vi "LSignal Numbering.vi"(8 "Signal Tag A":string[](array[string]), 9 "Selected L#":i32[](array[numeric]), 10 "Selected S IDX":i32[](array[numeric]), 11 "Signal Profile Table A":string[][](table) caption="Singla Profile Table") -> (0 "BS Table":string[][](table) caption="Singla Profile Table", 3 "L# for T":i32[](array[numeric]))   [LabVIEW 2018]
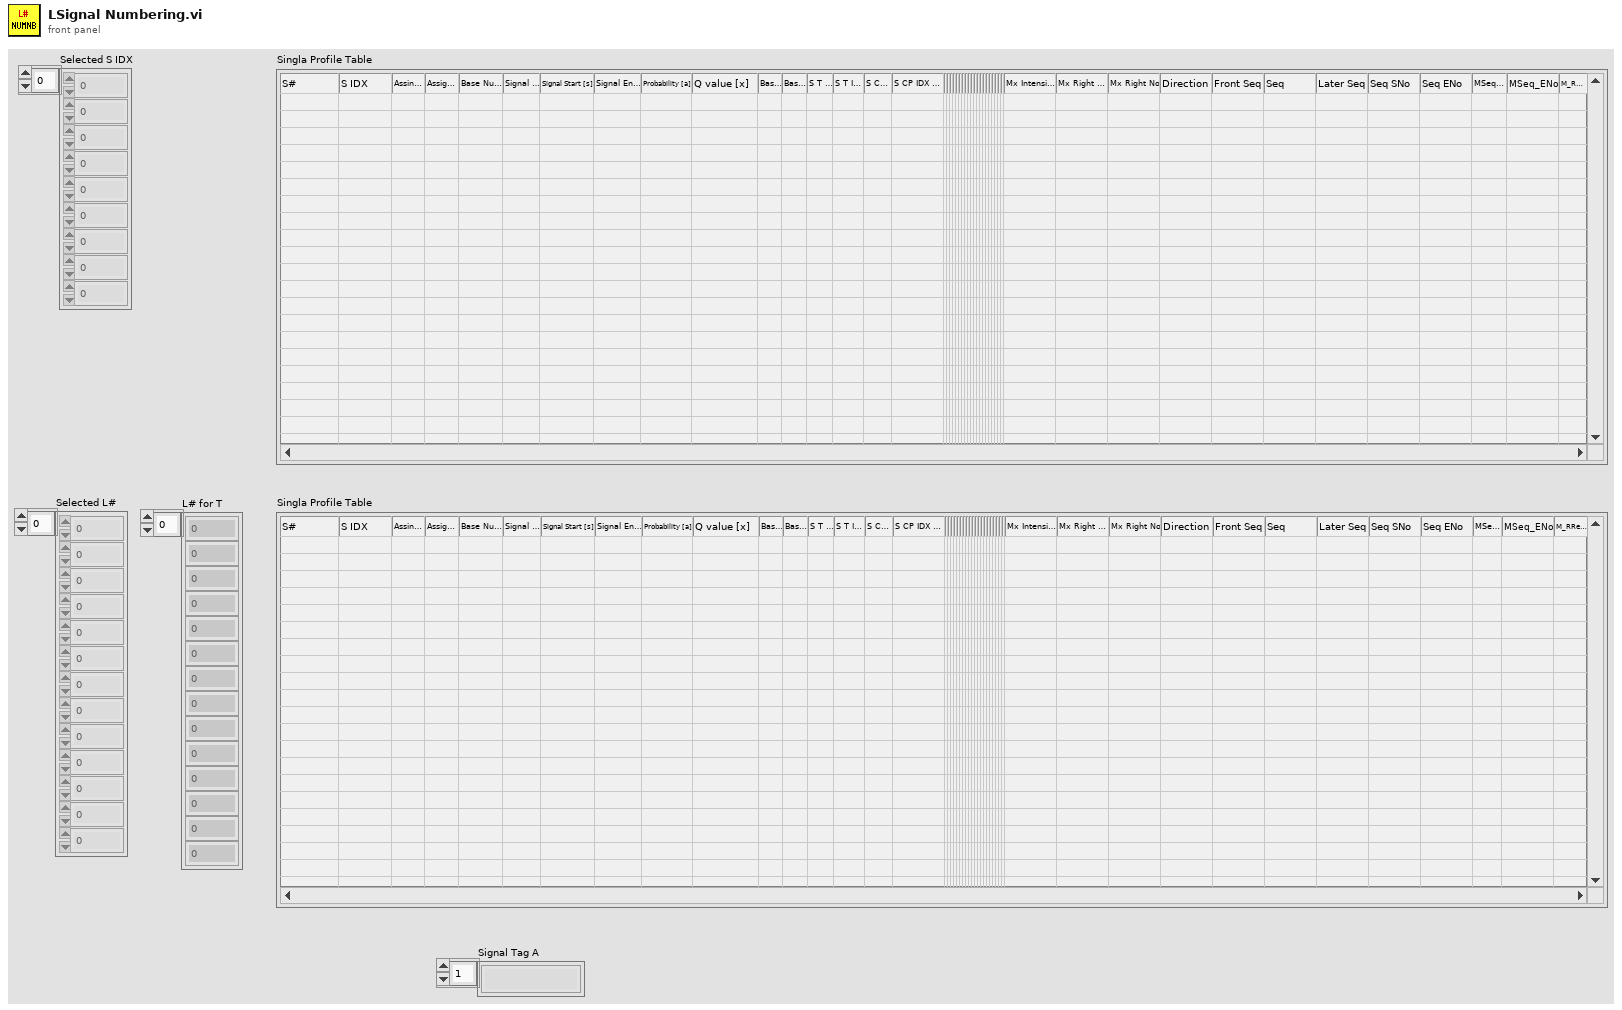
[diagram p1: front panel]
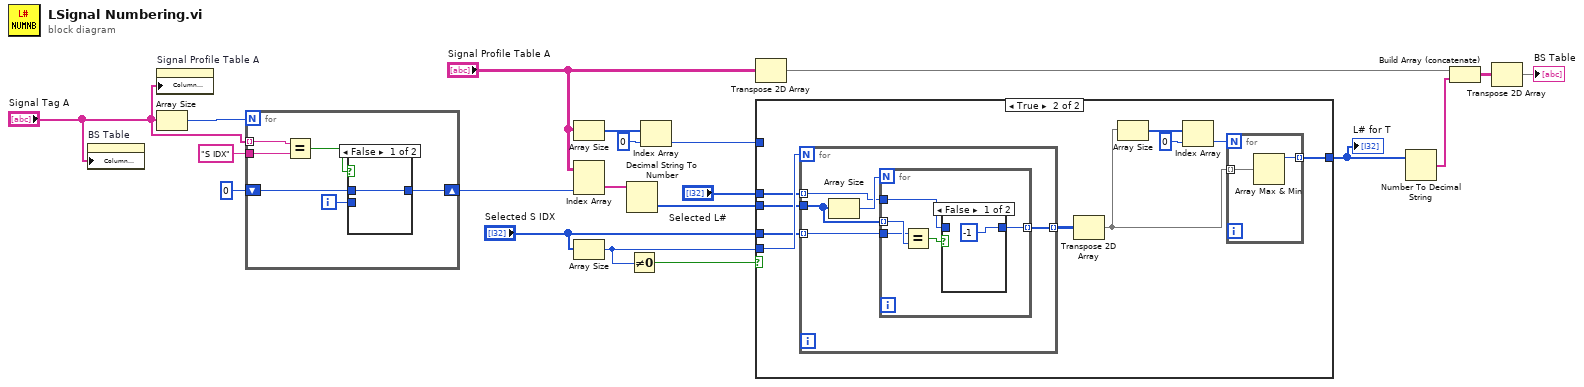
[diagram p0: block diagram]
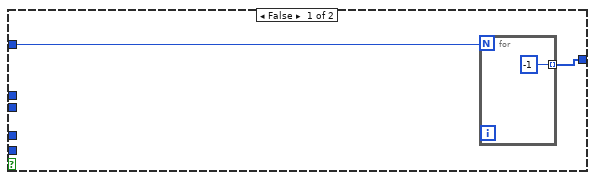
[diagram p2: hidden frame]
diagram:
  n1 = property on="BS Table" class="Tbl (strict)"("Column Headers[]"="Signal Tag A") -> ()  [unwired: 2 in, 2 out]
  n2 = property on="Signal Profile Table A" class="Tbl (strict)"("Column Headers[]"="Signal Tag A") -> ()  [unwired: 2 in, 2 out]
  n3 = Array Size(array="Signal Tag A") -> (size(s)=w15:i32)
  n4 = for {
    N: w15 -> [_]
    tunnel: "Signal Tag A" -> [w23] mode=indexing
    tunnel: "S IDX" ("グループ名入力") -> [w26]
    shift-right: [w21] -> w6
    shift-left: 0 -> [w25]
    i -> [w22]
    n5 = Equal?(x=w23, y=w26) -> (x = y?=w24:bool)
    n6 = case shown="False" w24 {
      tunnel: w22 -> [_ w28]
      tunnel: [w27 w28] -> w21
      tunnel: w25 -> [w27 _]
      frame False {
      }
      frame True {
      }
    }
  }
  n7 = Array Size(array="Signal Profile Table A") -> (size(s)=w20:i32[])
  n8 = Index Array(array="Signal Profile Table A", index (col)=w6) -> (element=w11:string[])  [unwired: 1 in]
  n9 = Array Size(array="Selected S IDX") -> (size(s)=w9:i32)
  n10 = Decimal String To Number(string=w11) -> (number=w7:i32[])  [unwired: 2 in, 1 out]
  n11 = Not Equal To 0?(x=w9) -> (x != 0?=w8:bool)
  n12 = Index Array(array=w20, index=0) -> (element=w5:i32)
  n13 = Transpose 2D Array(2D array="Signal Profile Table A") -> (transposed array=w2:string[][])
  n14 = case shown="True" w8 {
    tunnel: w9 -> [_ w41]
    tunnel: w7 -> [_ w39]
    tunnel: "Selected S IDX" -> [_ w40]
    tunnel: "Selected L#" -> [_ w34]
    tunnel: [w29 w32] -> w4
    tunnel: w5 -> [w30 _]
    frame False {
      n15 = for {
        N: w30 -> [_]
        tunnel: [-1] -> w29 mode=indexing
      }
    }
    frame True {
      n16 = for {
        N: w41 -> [_]
        tunnel: w40 -> [w46] mode=indexing
        tunnel: w39 -> [w47]
        tunnel: w34 -> [w45] mode=indexing
        tunnel: [w44] -> w33 mode=indexing
        n17 = Array Size(array=w47) -> (size(s)=w48:i32)
        n18 = for {
          N: w48 -> [_]
          tunnel: w47 -> [w53] mode=indexing
          tunnel: w46 -> [w52]
          tunnel: w45 -> [w50]
          tunnel: [w49] -> w44 mode=indexing
          n19 = Equal?(x=w52, y=w53) -> (x = y?=w51:bool)
          n20 = case shown="False" w51 {
            tunnel: w50 -> [_ w55]
            tunnel: [-1 w55] -> w49
            frame False {
            }
            frame True {
            }
          }
        }
      }
      n21 = Transpose 2D Array(2D array=w33) -> (transposed array=w35:i32[][])
      n22 = Array Size(array=w35) -> (size(s)=w38:i32[])
      n23 = Index Array(array=w38, index=0) -> (element=w36:i32)
      n24 = for {
        N: w36 -> [_]
        tunnel: w35 -> [w43] mode=indexing
        tunnel: [w42] -> w32 mode=indexing
        n25 = Array Max & Min(array=w43) -> (max value=w42:i32)  [unwired: 3 out]
      }
    }
  }
  "L# for T" <- w4
  n26 = Number To Decimal String(number=w4) -> (decimal integer string=w3:string[])  [unwired: 1 in]
  n27 = Build Array (concatenate)(w2, w3) -> (w17:string[][])
  n28 = Transpose 2D Array(2D array=w17) -> (transposed array=→"BS Table":string[][])
